vi "AO SCTR with Digital Out Engine.vi"(0 "Unique Notifier Name":string, 11 "AO PFI Lines":string[](array[string])) -> ()   [LabVIEW 2016]
uses:
  AO SCTR Type Defs/AO SCTR Notifier Type.ctl
  AO SCTR Type Defs/AO SCTR Actions.ctl
  <vilib>/DAQmx/write.llb/DAQmx Write (Analog DBL 1Chan 1Samp).vi
  <vilib>/Analysis/1siggen.llb/Ramp Pattern by Samples.vi
  <vilib>/DAQmx/write.llb/DAQmx Write (Analog 1D DBL 1Chan NSamp).vi
  <vilib>/DAQmx/create/channels.llb/DAQmx Create Channel (CO-Pulse Generation-Time).vi
  <vilib>/DAQmx/create/channels.llb/DAQmx Create Channel (AO-Voltage-Basic).vi
  <vilib>/DAQmx/miscellaneous.llb/DAQmx Fill In Error Info.vi
  <vilib>/DAQmx/configure/timing.llb/DAQmx Timing (Sample Clock).vi
  <resource>/objmgr/daqmx.rc
  <vilib>/Analysis/NI_AALBase.lvlib
panel:
  in  "Counter Idle State":i32(ring)=10214 items=["High"=10192, "Low"=10214]
  in  "Initial Delay":dbl format="%.6f"
  in  "Disable Input":bool
  out "Running":bool
  in  "Load":bool
  in  "Save":bool
  in  "Quit":bool
  in  "Waveform Settings":T1={"Actions"=enum."Stop at Offset", "Offset (V)"=-0.61, "Amplititude (V)"=0.524, "Samples Per Channel"=2280, "Start Delay (ms)"=20.0, "Running?"=FALSE, "Exposure Time (s)"=0.0} {"Amplititude (V)" format="%#_13g"; "Offset (V)" format="%#_13g"; "Start Delay (ms)" format="%#_13g"}
  out "Waveform Graph":dbl[](graph)
  out "Actual Sample Rate":dbl=10000.0 format="%0.2f"
  # "AO Line. Example: Dev1/ao1\nPFI (Trigger) Line. Example: /Dev1/PFI0\nCounter. Example: Dev1/ctr0"
  # "For debugging only."
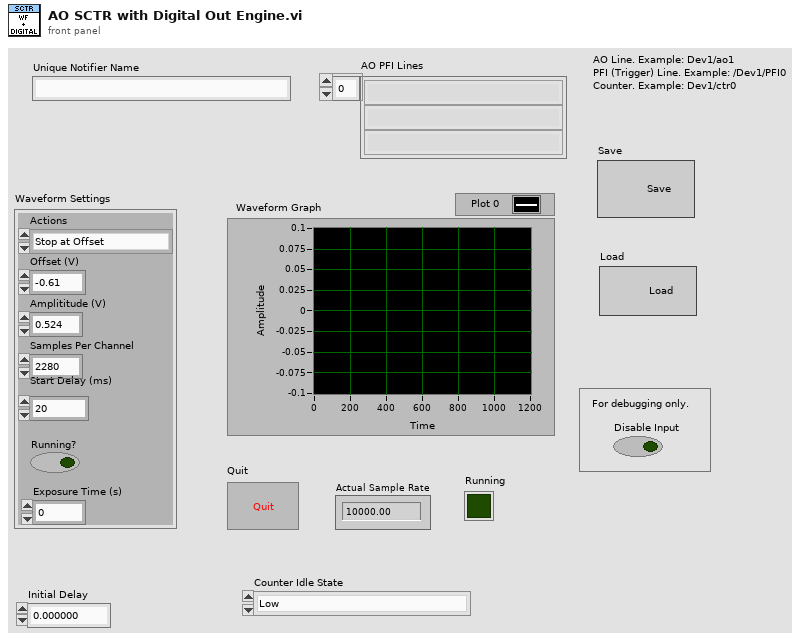
[diagram p1: front panel]
types:
  T1 = typedef "AO SCTR Notifier Type.ctl" = cluster{"Actions":T2, "Offset (V)":dbl, "Amplititude (V)":dbl, "Samples Per Channel":i32, "Start Delay (ms)":dbl, "Running?":bool, "Exposure Time (s)":dbl}
  T2 = typedef "AO SCTR Actions.ctl" = enum16{"Stop at Offset", "Update and Run", "Quit"}
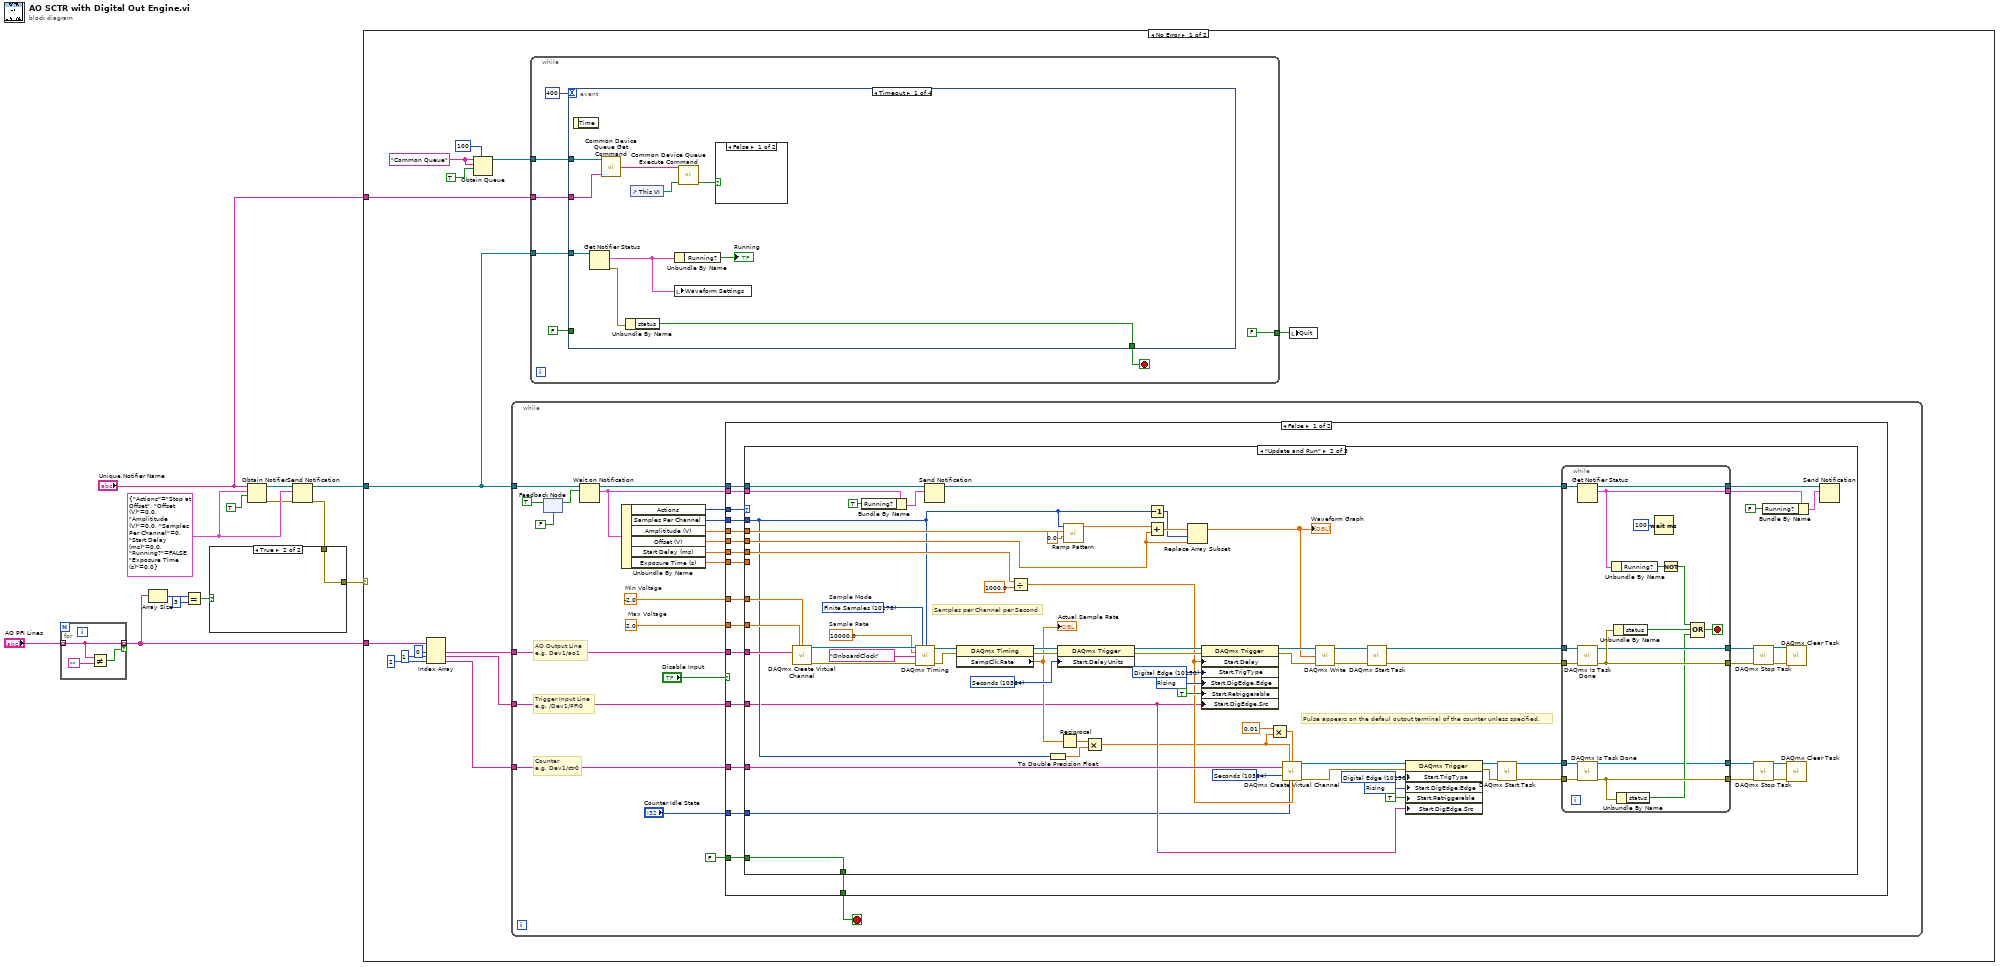
[diagram p0: block diagram]
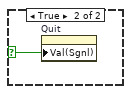
[diagram p2: hidden frame]
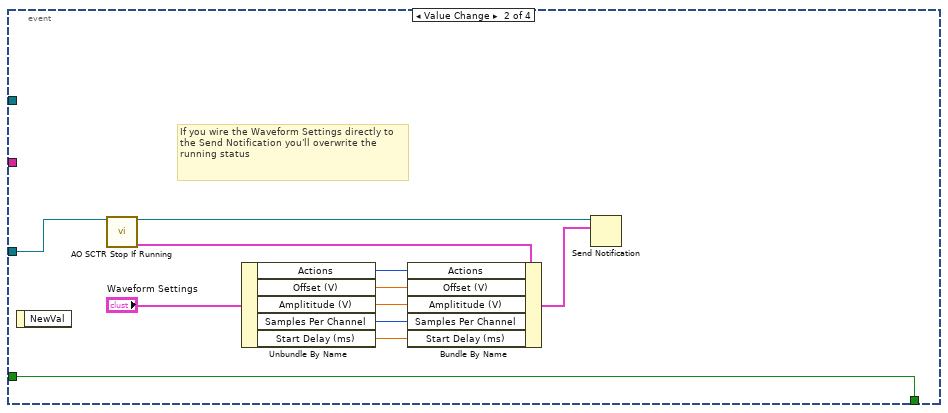
[diagram p3: hidden frame]
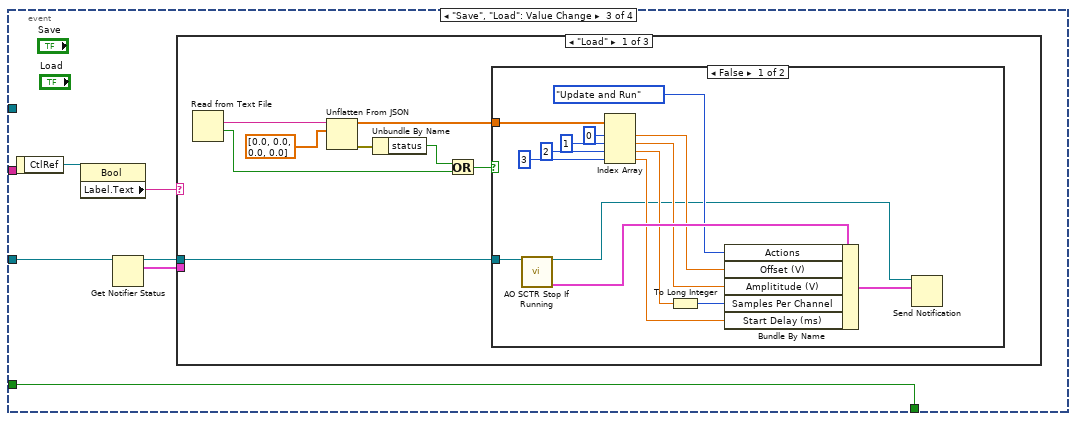
[diagram p4: hidden frame]
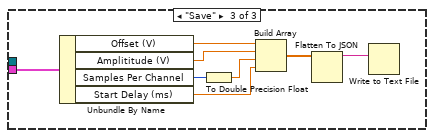
[diagram p7: hidden frame]
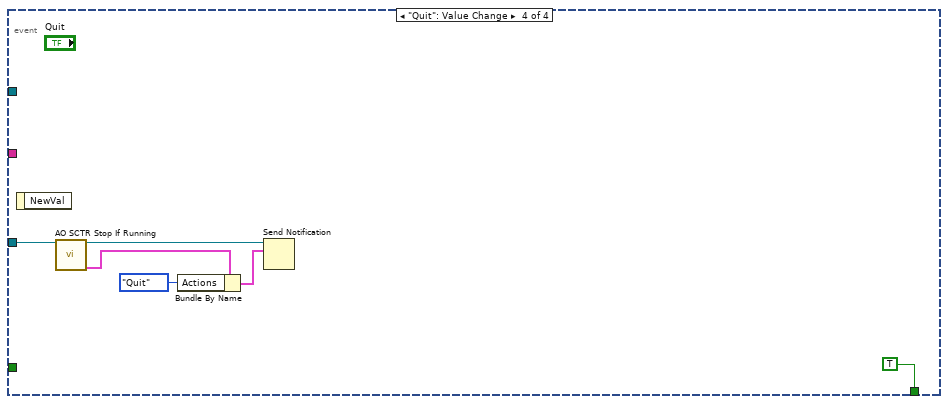
[diagram p8: hidden frame]
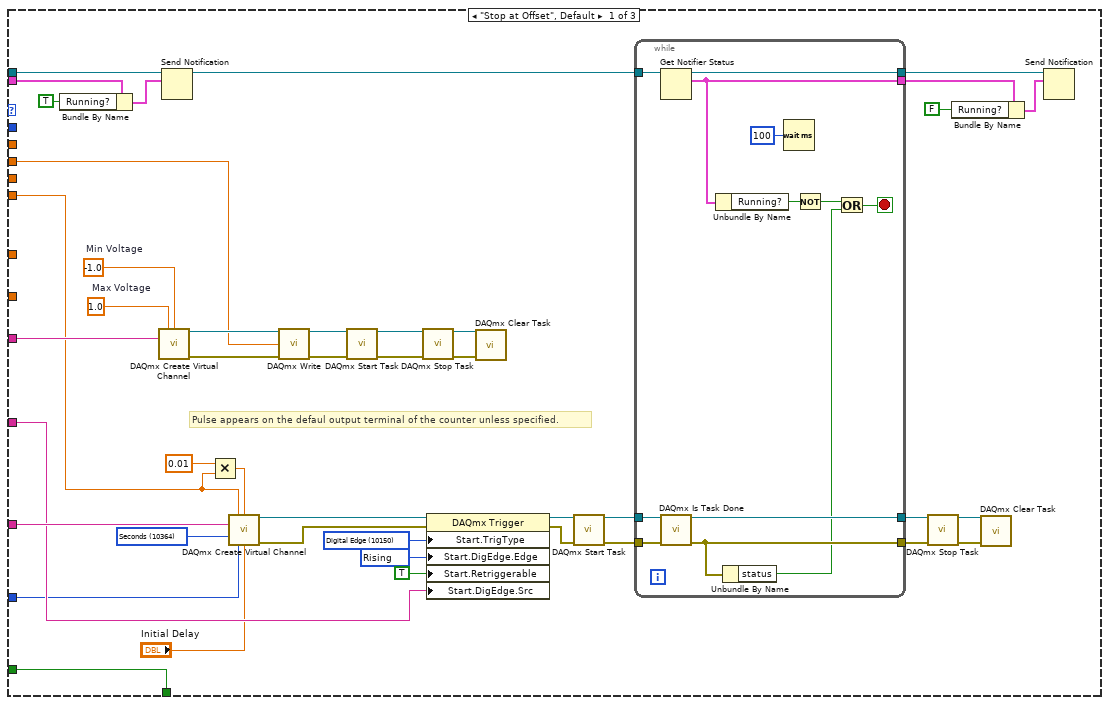
[diagram p9: hidden frame]
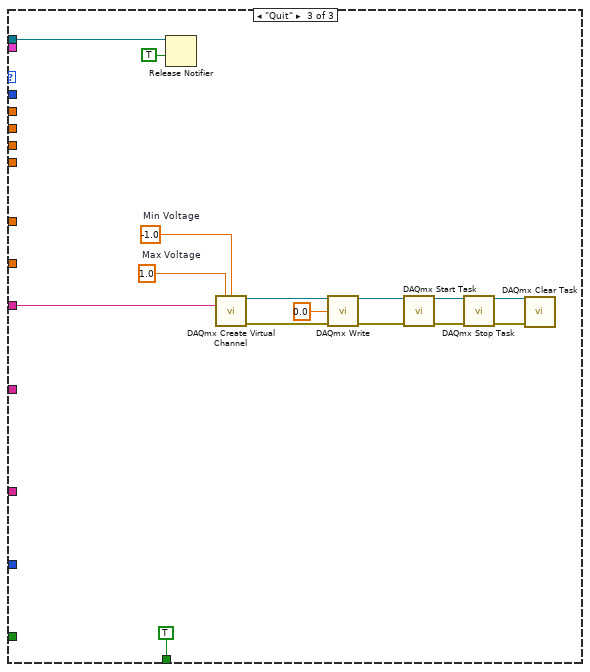
[diagram p10: hidden frame]
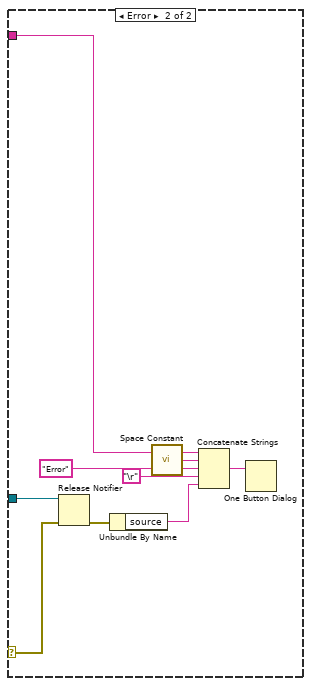
[diagram p12: hidden frame]
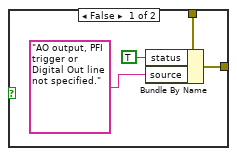
[diagram p13: hidden frame]
diagram:
  w8 = T1 {"Actions"=enum."Stop at Offset", "Offset (V)"=0.0, "Amplititude (V)"=0.0, "Samples Per Channel"=0, "Start Delay (ms)"=0.0, "Running?"=FALSE, "Exposure Time (s)"=0.0} ("Waveform Settings 2")
  n1 = for {
    tunnel: "AO PFI Lines" -> [w15] mode=indexing
    tunnel: [w15] -> w6 mode=indexing if=w14
    n2 = Not Equal?(x=w15, y="") -> (x != y?=w14:bool)
  }
  n3 = Array Size(array=w6) -> (size(s)=w5:i32)
  n4 = Equal?(x=w5, y=3) -> (x = y?=w3:bool)
  n5 = Obtain Notifier(name (unnamed)="Unique Notifier Name", notification data type=w8, create if not found? (T)=TRUE) -> (notifier out=w10:refnum<notifier>, error out=w7:errorcluster)  [unwired: 1 in, 1 out]
  n6 = Send Notification(notification=w8, notifier=w10, error in (no error)=w7) -> (notifier out=w9:refnum<notifier>, error out=w2:errorcluster)
  n7 = case shown="True" w3 {
    tunnel: w2 -> [w20 w21]
    tunnel: [w19 w21] -> w1
    frame False {
      n8 = Bundle By Name(cluster=w20, "status"=TRUE, "source"="AO output, PFI trigger or Digital Out line not specified.") -> (w19:errorcluster)
    }
    frame True {
    }
  }
  n9 = case shown="No Error" w1 {
    selector: w1 -> [_ w312]
    tunnel: "Unique Notifier Name" -> [w30 w310]
    tunnel: w9 -> [w25 w313]
    tunnel: w6 -> [w24 _]
    frame No Error {
      w35 = "Common Queue" ("Unique Notifier Name")
      n10 = Index Array(array=w24, index #1=0 ("index"), index #2=1 ("index"), index #3=2 ("index")) -> (element #1=w27:string, element #2=w26:string, element #3=w22:string)
      n11 = Obtain Queue(max queue size (-1, unlimited)=100, name (unnamed)=w35, element data type=w35, create if not found? (T)=TRUE) -> (queue out=w31:refnum<queue>)  [unwired: 1 in, 2 out]
      n12 = while {
        tunnel: w25 -> [w112]
        tunnel: w27 -> [w120]
        tunnel: w26 -> [w119]
        tunnel: w22 -> [w110]
        stop <- w121 stop-if-true
        w114 = 2.0  # Max Voltage
        w115 = -2.0  # Min Voltage
        # "Counter\ne.g. Dev1/ctr0"
        # "AO Output Line\ne.g. Dev1/ao1"
        # "Trigger Input Line\ne.g. /Dev1/PFI0"
        n13 = feedback-in #1(TRUE ("ignore previous (F)")) -> ()
        n14 = feedback #1(FALSE ("ignore previous (F)")) -> (w116:bool)
        n15 = Wait on Notification(notifier=w112, ignore previous (F)=w116) -> (notifier out=w123:refnum<notifier>, notification=w122:T1)  [unwired: 2 in, 2 out]
        n16 = Unbundle By Name(w122) -> ("Actions"=w124:T2, "Samples Per Channel"=w126:i32, "Amplititude (V)"=w128:dbl, "Offset (V)"=w125:dbl, "Start Delay (ms)"=w127:dbl, "Exposure Time (s)"=w109:dbl)
        n17 = case shown="False" "Disable Input" {
          tunnel: w128 -> [w144 _]
          tunnel: w127 -> [w143 _]
          tunnel: w126 -> [w142 _]
          tunnel: w125 -> [w141 _]
          tunnel: w124 -> [w140 _]
          tunnel: w123 -> [w139 _]
          tunnel: w122 -> [w138 _]
          tunnel: [w137 w304] -> w121
          tunnel: w120 -> [w136 _]
          tunnel: w119 -> [w135 _]
          tunnel: w115 -> [w134 _]
          tunnel: w114 -> [w133 _]
          tunnel: FALSE -> [w132 w304]
          tunnel: w110 -> [w131 _]
          tunnel: w109 -> [w130 _]
          tunnel: "Counter Idle State" -> [w129 _]
          frame False {
            n18 = case shown="\"Update and Run\"" w140 {
              tunnel: w144 -> [_ w246 _]
              tunnel: w143 -> [_ w229 _]
              tunnel: w142 -> [_ w216 _]
              tunnel: w141 -> [w177 w245 _]
              tunnel: w139 -> [w156 w244 w301]
              tunnel: w138 -> [w154 w242 _]
              tunnel: [w176 w236 TRUE] -> w137
              tunnel: w136 -> [w175 w239 w289]
              tunnel: w135 -> [w163 w205 _]
              tunnel: w134 -> [_ w238 _]
              tunnel: w133 -> [_ w237 _]
              tunnel: w132 -> [w176 w236 _]
              tunnel: w131 -> [w164 w225 _]
              tunnel: w130 -> [w146 _ _]
              tunnel: w129 -> [w145 w200 _]
              frame "Stop at Offset", Default {
                w172 = 10280 items=["Rising"=10280, "Falling"=10171] ("Start.DigEdge.Edge")
                w173 = 10150 items=["Analog Edge"=10099, "Analog Multi Edge"=16108, "Digital Edge"=10150, "Digital Pattern"=10398, "Analog Window"=10103, "Time"=15996, "None"=10230] ("Start.TrigType")
                w174 = 10364 items=["Seconds"=10364] ("units")
                w179 = 1.0  # Max Voltage
                w178 = -1.0  # Min Voltage
                # "Pulse appears on the defaul output terminal of the counter unless specified."
                n19 = Bundle By Name(cluster=w154, "Running?"=TRUE ("Running")) -> (w157:T1)
                n20 = call-poly <vilib>:"DAQmx Create Virtual Channel.vi"("maximum value"=w179, "minimum value"=w178, "physical channels"=w175) -> ("task out"=w180:refnum<k21>, "error out"=w185:errorcluster)  [unwired: 11 in]
                n21 = Send Notification(notification=w157, notifier=w156) -> (notifier out=w155:refnum<notifier>)  [unwired: 1 in, 1 out]
                n22 = Multiply(x=0.01, y=w146) -> (x*y=w148:dbl)
                n23 = call-poly <vilib>:"DAQmx Create Virtual Channel.vi"("high time"=w146, "low time"=w148, "counter"=w164, "units"=w174, "idle state"=w145, "initial delay"="Initial Delay") -> ("task out"=w166:refnum<k21>, "error out"=w165:errorcluster)  [unwired: 8 in]
                n24 = call-poly <vilib>:"DAQmx Write.vi"("task/channels in"=w180, "data"=w177, "error in"=w185) -> ("task out"=w181:refnum<k21>, "error out"=w186:errorcluster)  [unwired: 10 in, 1 out]
                n25 = call <vilib>:"DAQmx Start Task.vi"("task/channels in"=w181, "error in"=w186) -> ("task out"=w183:refnum<k21>, "error out"=w187:errorcluster)  [unwired: 12 in]
                n26 = call <vilib>:"DAQmx Stop Task.vi"("task/channels in"=w183, "error in"=w187) -> ("task out"=w184:refnum<k21>, "error out"=w182:errorcluster)  [unwired: 12 in]
                n27 = property class="DAQmx Trigger"(reference=w166, error in=w165, "Start.TrigType"=w173, "Start.DigEdge.Edge"=w172, "Start.Retriggerable"=TRUE, "Start.DigEdge.Src"=w163) -> (reference out=w170:refnum<k21>, error out=w169:errorcluster)
                n28 = call <vilib>:"DAQmx Clear Task.vi"("task in"=w184, "error in"=w182) -> ()  [unwired: 13 in, 1 out]
                n29 = call <vilib>:"DAQmx Start Task.vi"("task/channels in"=w170, "error in"=w169) -> ("task out"=w160:refnum<k21>, "error out"=w159:errorcluster)  [unwired: 12 in]
                n30 = while {
                  tunnel: w155 -> [w199]
                  tunnel: w159 -> [w195]
                  tunnel: w160 -> [w196]
                  tunnel: [w194] -> w161
                  tunnel: [w193] -> w162
                  tunnel: [w189] -> w151
                  tunnel: [w188] -> w150
                  stop <- w190 stop-if-true
                  n31 = Get Notifier Status(notifier=w199) -> (notifier out=w189:refnum<notifier>, current notification=w188:T1)  [unwired: 1 in, 3 out]
                  n32 = call <vilib>:"DAQmx Is Task Done.vi"("task/channels in"=w196, "error in"=w195) -> ("task out"=w193:refnum<k21>, "error out"=w194:errorcluster)  [unwired: 11 in, 1 out]
                  n33 = Unbundle By Name(w188) -> ("Running?"=w198:bool)
                  n34 = Unbundle By Name(w194) -> ("status"=w191:bool)
                  n35 = Wait (ms)(milliseconds to wait=u32 100) -> ()  [unwired: 1 out]
                  n36 = Not(x=w198) -> (.not. x?=w192:bool)
                  n37 = Or(x=w192, y=w191) -> (x .or. y?=w190:bool)
                }
                n38 = call <vilib>:"DAQmx Stop Task.vi"("task/channels in"=w162, "error in"=w161) -> ("task out"=w167:refnum<k21>, "error out"=w168:errorcluster)  [unwired: 12 in]
                n39 = Bundle By Name(cluster=w150, "Running?"=FALSE ("Running")) -> (w152:T1)
                n40 = call <vilib>:"DAQmx Clear Task.vi"("task in"=w167, "error in"=w168) -> ()  [unwired: 13 in, 1 out]
                n41 = Send Notification(notification=w152, notifier=w151) -> ()  [unwired: 1 in, 2 out]
              }
              frame "Update and Run" {
                w221 = 10280 items=["Rising"=10280, "Falling"=10171] ("Start.DigEdge.Edge")
                w222 = 10150 items=["Analog Edge"=10099, "Analog Multi Edge"=16108, "Digital Edge"=10150, "Digital Pattern"=10398, "Analog Window"=10103, "Time"=15996, "None"=10230] ("Start.TrigType")
                w223 = 10364 items=["Seconds"=10364] ("units")
                w231 = 10364 items=["Sample Clock Periods"=10286, "Seconds"=10364, "Ticks"=10304] ("Start.DelayUnits")
                w264 = 10000.0  # Sample Rate
                w256 = 10280 items=["Rising"=10280, "Falling"=10171] ("Start.DigEdge.Edge")
                w247 = 10150 items=["Analog Edge"=10099, "Digital Edge"=10150, "Digital Pattern"=10398, "Analog Window"=10103, "None"=10230] ("Start.TrigType")
                w270 = 10178 items=["Finite Samples"=10178, "Continuous Samples"=10123, "Hardware Timed Single Point"=12522]  # Sample Mode
                # "Pulse appears on the defaul output terminal of the counter unless specified."
                # "Samples per Channel per Second"
                n42 = call-poly <vilib>:"DAQmx Create Virtual Channel.vi"("maximum value"=w237, "minimum value"=w238, "physical channels"=w239) -> ("task out"=w268:refnum<k21>, "error out"=w269:errorcluster)  [unwired: 11 in]
                n43 = Bundle By Name(cluster=w242, "Running?"=TRUE ("Running")) -> (w240:T1)
                n44 = call-poly <vilib>:"DAQmx Timing.vi"("task/channels in"=w268, "sample mode"=w270, "samples per channel"=w216, "rate"=w264, "source"=tag "OnboardClock" ("Sample Clock Source"), "error in"=w269) -> ("task out"=w254:refnum<k21>, "error out"=w271:errorcluster)  [unwired: 8 in]
                n45 = Send Notification(notification=w240, notifier=w244) -> (notifier out=w243:refnum<notifier>)  [unwired: 1 in, 1 out]
                n46 = property class="DAQmx Timing"(reference=w254, error in=w271) -> (reference out=w230:refnum<k21>, error out=w226:errorcluster, "SampClk.Rate"=w218:dbl)
                "Actual Sample Rate" <- w218
                n47 = Divide(x=w229, y=1000.0) -> (x/y=w219:dbl)
                n48 = To Double Precision Float(number=w216) -> (double precision float=w215:dbl)
                n49 = property class="DAQmx Trigger"(reference=w230, error in=w226, "Start.DelayUnits"=w231) -> (reference out=w224:refnum<k21>, error out=w227:errorcluster)
                n50 = Reciprocal(x=w218) -> (1/x=w217:dbl)
                n51 = call-poly <vilib>:"Ramp Pattern.vi"("start"=0.0, "end"=w246, "samples"=w216) -> ("Ramp Pattern"=w251:dbl[])  [unwired: 7 in, 1 out]
                n52 = Multiply(x=w217, y=w215) -> (x*y=w204:dbl)
                n53 = Decrement(x=w216) -> (x-1=w249:i32)
                n54 = Add(x=w251, y=w245) -> (x+y=w250:dbl[])
                n55 = Replace Array Subset(array=w250, new element=w245, index=w249) -> (w248:dbl[])
                "Waveform Graph" <- w248
                n56 = property class="DAQmx Trigger"(reference=w224, error in=w227, "Start.Delay"=w219, "Start.TrigType"=w247, "Start.DigEdge.Edge"=w256, "Start.Retriggerable"=TRUE, "Start.DigEdge.Src"=w205) -> (reference out=w257:refnum<k21>, error out=w252:errorcluster)
                n57 = Multiply(x=0.01, y=w204) -> (x*y=w203:dbl)
                n58 = call-poly <vilib>:"DAQmx Create Virtual Channel.vi"("high time"=w204, "low time"=w203, "counter"=w225, "units"=w223, "idle state"=w200, "initial delay"=w219) -> ("task out"=w202:refnum<k21>, "error out"=w201:errorcluster)  [unwired: 8 in]
                n59 = call-poly <vilib>:"DAQmx Write.vi"("task/channels in"=w257, "data"=w248, "error in"=w252) -> ("task out"=w263:refnum<k21>, "error out"=w262:errorcluster)  [unwired: 10 in, 1 out]
                n60 = call <vilib>:"DAQmx Start Task.vi"("task/channels in"=w263, "error in"=w262) -> ("task out"=w267:refnum<k21>, "error out"=w266:errorcluster)  [unwired: 12 in]
                n61 = property class="DAQmx Trigger"(reference=w202, error in=w201, "Start.TrigType"=w222, "Start.DigEdge.Edge"=w221, "Start.Retriggerable"=TRUE, "Start.DigEdge.Src"=w205) -> (reference out=w213:refnum<k21>, error out=w212:errorcluster)
                n62 = call <vilib>:"DAQmx Start Task.vi"("task/channels in"=w213, "error in"=w212) -> ("task out"=w210:refnum<k21>, "error out"=w211:errorcluster)  [unwired: 12 in]
                n63 = while {
                  tunnel: w267 -> [w288]
                  tunnel: w266 -> [w287]
                  tunnel: [w286] -> w258
                  tunnel: [w285] -> w259
                  tunnel: w243 -> [w284]
                  tunnel: [w282] -> w235
                  tunnel: [w281] -> w232
                  tunnel: w211 -> [w278]
                  tunnel: w210 -> [w279]
                  tunnel: [w277] -> w206
                  tunnel: [w272] -> w207
                  stop <- w273 stop-if-true
                  n64 = Get Notifier Status(notifier=w284) -> (notifier out=w282:refnum<notifier>, current notification=w281:T1)  [unwired: 1 in, 3 out]
                  n65 = call <vilib>:"DAQmx Is Task Done.vi"("task/channels in"=w288, "error in"=w287) -> ("task out"=w285:refnum<k21>, "error out"=w286:errorcluster)  [unwired: 11 in, 1 out]
                  n66 = call <vilib>:"DAQmx Is Task Done.vi"("task/channels in"=w279, "error in"=w278) -> ("task out"=w272:refnum<k21>, "error out"=w277:errorcluster)  [unwired: 11 in, 1 out]
                  n67 = Unbundle By Name(w281) -> ("Running?"=w283:bool)
                  n68 = Unbundle By Name(w286) -> ("status"=w276:bool)
                  n69 = Unbundle By Name(w277) -> ("status"=w274:bool)
                  n70 = Wait (ms)(milliseconds to wait=u32 100) -> ()  [unwired: 1 out]
                  n71 = Not(x=w283) -> (.not. x?=w275:bool)
                  n72 = Compound Arithmetic op=OR(w275, w276, w274) -> (w273:bool)
                }
                n73 = call <vilib>:"DAQmx Stop Task.vi"("task/channels in"=w259, "error in"=w258) -> ("task out"=w261:refnum<k21>, "error out"=w260:errorcluster)  [unwired: 12 in]
                n74 = call <vilib>:"DAQmx Stop Task.vi"("task/channels in"=w207, "error in"=w206) -> ("task out"=w208:refnum<k21>, "error out"=w209:errorcluster)  [unwired: 12 in]
                n75 = Bundle By Name(cluster=w232, "Running?"=FALSE ("Running")) -> (w233:T1)
                n76 = call <vilib>:"DAQmx Clear Task.vi"("task in"=w261, "error in"=w260) -> ()  [unwired: 13 in, 1 out]
                n77 = call <vilib>:"DAQmx Clear Task.vi"("task in"=w208, "error in"=w209) -> ()  [unwired: 13 in, 1 out]
                n78 = Send Notification(notification=w233, notifier=w235) -> ()  [unwired: 1 in, 2 out]
              }
              frame "Quit" {
                w292 = 1.0  # Max Voltage
                w291 = -1.0  # Min Voltage
                n79 = Release Notifier(notifier=w301, force destroy? (F)=TRUE) -> ()  [unwired: 1 in, 3 out]
                n80 = call-poly <vilib>:"DAQmx Create Virtual Channel.vi"("maximum value"=w292, "minimum value"=w291, "physical channels"=w289) -> ("task out"=w293:refnum<k21>, "error out"=w298:errorcluster)  [unwired: 11 in]
                n81 = call-poly <vilib>:"DAQmx Write.vi"("task/channels in"=w293, "data"=0.0, "error in"=w298) -> ("task out"=w294:refnum<k21>, "error out"=w299:errorcluster)  [unwired: 10 in, 1 out]
                n82 = call <vilib>:"DAQmx Start Task.vi"("task/channels in"=w294, "error in"=w299) -> ("task out"=w296:refnum<k21>, "error out"=w300:errorcluster)  [unwired: 12 in]
                n83 = call <vilib>:"DAQmx Stop Task.vi"("task/channels in"=w296, "error in"=w300) -> ("task out"=w297:refnum<k21>, "error out"=w295:errorcluster)  [unwired: 12 in]
                n84 = call <vilib>:"DAQmx Clear Task.vi"("task in"=w297, "error in"=w295) -> ()  [unwired: 13 in, 1 out]
              }
            }
          }
          frame True {
          }
        }
      }
      n85 = while {
        tunnel: w25 -> [w42]
        tunnel: [FALSE] -> w32
        tunnel: w31 -> [w38]
        tunnel: w30 -> [w37]
        stop <- w40 stop-if-true
        n86 = event shown="[0] Timeout" {
          selector: _ -> [_ _ _ _]
          dyn-events: _ -> [_ _ _ _]
          timeout: 400 -> [_ _ _ _]
          tunnel: w42 -> [w52 w63 w68 w104]
          tunnel: [w50 w64 w65 TRUE ("status")] -> w40
          tunnel: w38 -> [w46 _ _ _]
          tunnel: w37 -> [w45 _ _ _]
          tunnel: FALSE ("status") -> [_ w64 w65 _]
          event Timeout {
            n87 = event-data() -> ()  [unwired: 1 in, 1 out]
            n88 = Get Notifier Status(notifier=w52) -> (current notification=w43:T1, error out=w51:errorcluster)  [unwired: 1 in, 3 out]
            n89 = call "Common Device Queue Get Command.vi"("Common Queue"=w46, "Notifier Name"=w45) -> ("Command"=w48:string)  [unwired: 12 in, 1 out]
            n90 = Unbundle By Name(w51) -> ("status"=w50:bool)
            n91 = control-ref of="This VI"() -> (w47:refnum<vi>)
            n92 = Unbundle By Name(w43) -> ("Running?"=→"Running":bool)
            n93 = local write "Waveform Settings"(w43) -> ()
            n94 = call "Common Device Queue Execute Command.vi"("Common Command"=w48, "VI Refnum"=w47) -> ("Quit?"=w49:bool)  [unwired: 12 in, 1 out]
            n95 = case shown="False" w49 {
              selector: w49 -> [_ w53]
              frame False {
              }
              frame True {
                n96 = property on="Quit" class="Bool (strict)"("Val(Sgnl)"=w53) -> ()  [unwired: 2 in, 2 out]
              }
            }
          }
          event Value Change {
            # "If you wire the Waveform Settings directly to the Send Notification you'll overwrite the running status"
            n97 = event-data() -> ()  [unwired: 1 in, 1 out]
            n98 = call "AO SCTR Stop If Running.vi"("AO SCTR Notifier"=w63) -> ("AO SCTR Notifier (Dup)"=w62:refnum<notifier>, "Latest Notification"=w61:T1)  [unwired: 13 in]
            n99 = Unbundle By Name("Waveform Settings") -> ("Actions"=w58:T2, "Offset (V)"=w57:dbl, "Amplititude (V)"=w56:dbl, "Samples Per Channel"=w55:i32, "Start Delay (ms)"=w54:dbl)
            n100 = Bundle By Name(cluster=w61, "Actions"=w58, "Offset (V)"=w57, "Amplititude (V)"=w56, "Samples Per Channel"=w55, "Start Delay (ms)"=w54) -> (w60:T1)
            n101 = Send Notification(notification=w60, notifier=w62) -> ()  [unwired: 1 in, 2 out]
          }
          event "Save", "Load": Value Change {
            n102 = event-data() -> ("CtlRef"=w70:refnum<vi>)  [unwired: 1 in]
            n103 = property class="Bool"(reference=w70) -> ("Label.Text"=w69:string)  [unwired: 1 in, 2 out]
            n104 = Get Notifier Status(notifier=w68) -> (notifier out=w66:refnum<notifier>, current notification=w67:T1)  [unwired: 1 in, 3 out]
            n105 = case shown="\"Load\"" w69 {
              tunnel: w67 -> [_ _ w101]
              tunnel: w66 -> [w72 _ _]
              frame "Load" {
                n106 = Read from Text File() -> (text=w78:string, cancelled=w74:bool)  [unwired: 4 in, 2 out]
                n107 = Unflatten From JSON(JSON string=w78, type and defaults=dbl[] [0.0, 0.0, 0.0, 0.0]) -> (value=w71:dbl[], error out=w76:errorcluster)  [unwired: 5 in]
                n108 = Unbundle By Name(w76) -> ("status"=w75:bool)
                n109 = Or(x=w75, y=w74) -> (x .or. y?=w73:bool)
                n110 = case shown="False" w73 {
                  tunnel: w72 -> [w93 _]
                  tunnel: w71 -> [w90 _]
                  frame False {
                    n111 = call "AO SCTR Stop If Running.vi"("AO SCTR Notifier"=w93) -> ("AO SCTR Notifier (Dup)"=w80:refnum<notifier>, "Latest Notification"=w92:T1)  [unwired: 13 in]
                    n112 = Index Array(array=w90, index #1=0 ("index"), index #2=1 ("index"), index #3=2 ("index"), index #4=3 ("index")) -> (element #1=w81:dbl, element #2=w82:dbl, element #3=w84:dbl, element #4=w85:dbl)
                    n113 = To Long Integer(number=w84) -> (32bit integer=w83:i32)
                    n114 = Bundle By Name(cluster=w92, "Actions"=AO_SCTR_Actions."Update and Run", "Offset (V)"=w81, "Amplititude (V)"=w82, "Samples Per Channel"=w83, "Start Delay (ms)"=w85) -> (w79:T1)
                    n115 = Send Notification(notification=w79, notifier=w80) -> ()  [unwired: 1 in, 2 out]
                  }
                  frame True {
                  }
                }
              }
              frame Default {
              }
              frame "Save" {
                n116 = Unbundle By Name(w101) -> ("Offset (V)"=w100:dbl, "Amplititude (V)"=w97:dbl, "Samples Per Channel"=w98:i32, "Start Delay (ms)"=w99:dbl)
                n117 = To Double Precision Float(number=w98) -> (double precision float=w96:dbl)
                n118 = Build Array(w100, w97, w96, w99) -> (w95:dbl[])
                n119 = Flatten To JSON(anything=w95) -> (JSON string=w94:string)  [unwired: 2 in, 1 out]
                n120 = Write to Text File(text=w94) -> ()  [unwired: 3 in, 3 out]
              }
            }
          }
          event "Quit": Value Change {
            n121 = event-data() -> ()  [unwired: 1 in, 1 out]
            n122 = call "AO SCTR Stop If Running.vi"("AO SCTR Notifier"=w104) -> ("AO SCTR Notifier (Dup)"=w103:refnum<notifier>, "Latest Notification"=w102:T1)  [unwired: 13 in]
            n123 = Bundle By Name(cluster=w102, "Actions"=AO_SCTR_Actions."Quit") -> (w106:T1)
            n124 = Send Notification(notification=w106, notifier=w103) -> ()  [unwired: 1 in, 2 out]
          }
        }
      }
      n125 = local write "Quit"(w32) -> ()
    }
    frame Error {
      n126 = Release Notifier(notifier=w313, error in (no error)=w312) -> (error out=w306:errorcluster)  [unwired: 1 in, 2 out]
      n127 = Unbundle By Name(w306) -> ("source"=w305:string)
      n128 = call <vilib>:"Space Constant.vi"() -> ("String"=w309:string)
      n129 = Concatenate Strings(w310, w309, "Error" ("string"), "\r", w305) -> (w311:string)
      n130 = One Button Dialog(message=w311) -> ()  [unwired: 1 in, 1 out]
    }
  }
